vi "Create Controls in Configuration.vi"(8 "error in":errorcluster, 9 "vi refnum":refnum<vi>, 10 "control refnum in":refnum<vi>, 11 "cluster ref":refnum<vi>) -> (0 "error out":errorcluster, 3 "control refnum out":refnum<vi>)   [LabVIEW 2021, in "Converter.lvlib"]
uses:
  Converter.lvlib
  <vilib>/Utility/miscctls.llb/LVPositionTypeDef.ctl
  <vilib>/numeric/LVNumericRepresentation.ctl
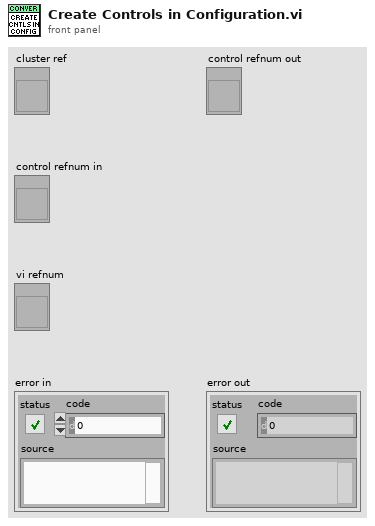
[diagram p1: front panel]
types:
  T1 = typedef "LVPositionTypeDef.ctl" = cluster{"Left":i32, "Top":i32}
  T2 = typedef "LVNumericRepresentation.ctl" = enum32{"Extended Precision", "Double Precision", "Single Precision", "Long", "Word", "Byte", "Unsigned Long", "Unsigned Word", "Unsigned Byte", "Complex Extended", "Complex Double", "Complex Single", "Quad", "Unsigned Quad", "Fixed-Point"}
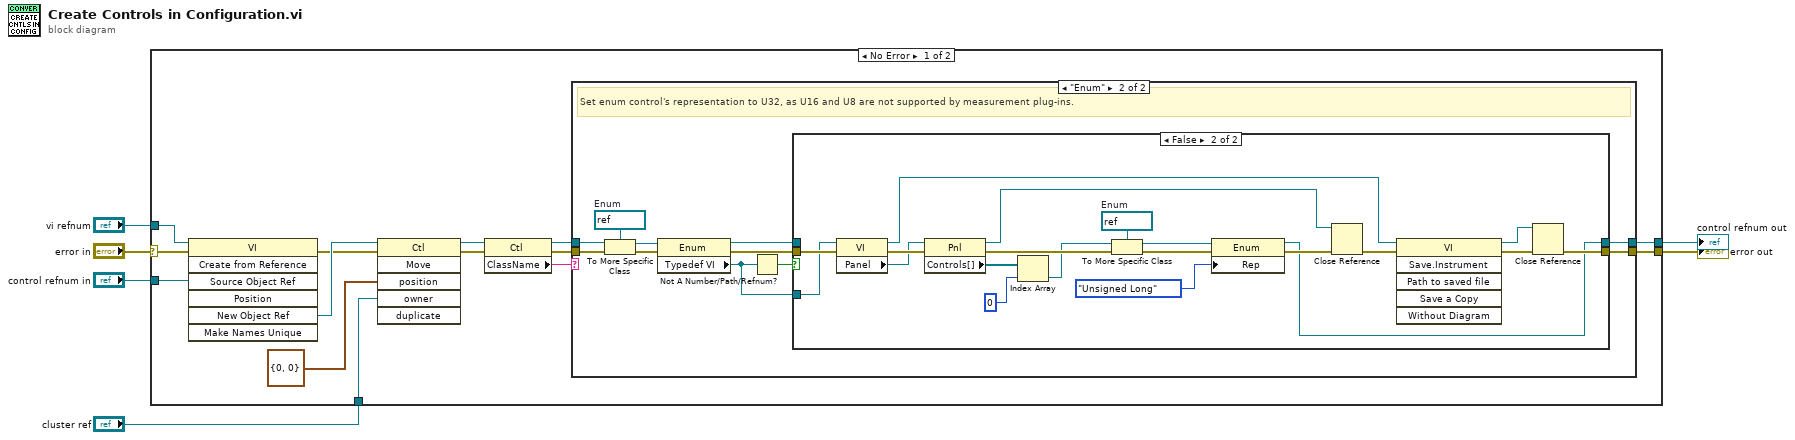
[diagram p0: block diagram]
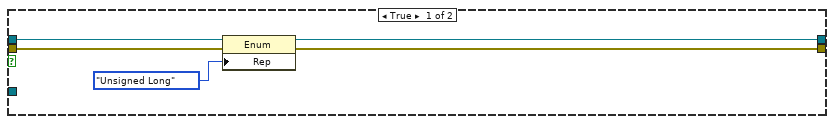
[diagram p3: hidden frame]
diagram:
  n1 = case shown="No Error" "error in" {
    selector: "error in" -> [w18 w59]
    tunnel: [w11 w59] -> w1
    tunnel: "control refnum in" -> [w20 _]
    tunnel: "cluster ref" -> [w7 _]
    tunnel: "vi refnum" -> [w19 _]
    tunnel: [w8 _] -> w2
    frame No Error {
      n2 = invoke class="VI" method="Create from Reference"(reference=w19, error in=w18, "Source Object Ref"=w20) -> (error out=w15:errorcluster, "New Object Ref"=w16:refnum<vi>)  [unwired: 4 in, 5 out]
      n3 = invoke class="Ctl" method="Move"(reference=w16, error in=w15, "position"=T1 {"Left"=0, "Top"=0}, "owner"=w7) -> (reference out=w13:refnum<vi>, error out=w14:errorcluster)  [unwired: 2 in, 4 out]
      n4 = property class="Ctl"(reference=w13, error in=w14) -> (reference out=w9:refnum<vi>, error out=w12:errorcluster, "ClassName"=w10:string)
      n5 = case shown="\"Enum\"" w10 {
        tunnel: [w22 w28] -> w11
        tunnel: w12 -> [w22 w33]
        tunnel: w9 -> [w21 w32]
        tunnel: [w21 w27] -> w8
        frame Default {
        }
        frame "Enum" {
          w31 = refnum<vi> refnum  # Enum
          # "Set enum control's representation to U32, as U16 and U8 are not supported by measurement plug-ins."
          n6 = To More Specific Class(target class=w31, reference=w32, error in=w33) -> (specific class reference=w26:refnum<vi>, error out=w25:errorcluster)
          n7 = property class="Enum"(reference=w26, error in=w25) -> (reference out=w29:refnum<vi>, error out=w30:errorcluster, "Typedef VI"=w23:refnum<vi>)
          n8 = Not A Number/Path/Refnum?(number/path/refnum=w23) -> (NaN/Path/Refnum?=w24:bool)
          n9 = case shown="False" w24 {
            tunnel: w30 -> [w38 w58]
            tunnel: w29 -> [w36 _]
            tunnel: [w37 w43] -> w28
            tunnel: [w35 w39] -> w27
            tunnel: w23 -> [_ w56]
            frame True {
              n10 = property class="Enum"(reference=w36, error in=w38, "Rep"=LVNumericRepresentation."Unsigned Long" ("Representation")) -> (reference out=w35:refnum<vi>, error out=w37:errorcluster)
            }
            frame False {
              w49 = refnum<vi> refnum  # Enum
              n11 = property class="VI"(reference=w56, error in=w58) -> (reference out=w41:refnum<vi>, error out=w57:errorcluster, "Panel"=w54:refnum<vi>)
              n12 = property class="Pnl"(reference=w54, error in=w57) -> (reference out=w44:refnum<vi>, error out=w55:errorcluster, "Controls[]"=w46:refnum<vi>[])
              n13 = Index Array(array=w46, index=0) -> (element=w51:refnum<vi>)
              n14 = To More Specific Class(target class=w49, reference=w51, error in=w55) -> (specific class reference=w50:refnum<vi>, error out=w52:errorcluster)
              n15 = property class="Enum"(reference=w50, error in=w52, "Rep"=LVNumericRepresentation."Unsigned Long" ("Representation")) -> (reference out=w39:refnum<vi>, error out=w47:errorcluster)
              n16 = Close Reference(reference=w44, error in (no error)=w47) -> (error out=w45:errorcluster)
              n17 = invoke class="VI" method="Save.Instrument"(reference=w41, error in=w45) -> (reference out=w40:refnum<vi>, error out=w42:errorcluster)  [unwired: 4 in, 4 out]
              n18 = Close Reference(reference=w40, error in (no error)=w42) -> (error out=w43:errorcluster)
            }
          }
        }
      }
    }
    frame Error {
    }
  }
  "control refnum out" <- w2
  "error out" <- w1
